vi "log.vi"(8 "error in (no error)":errorcluster, 10 "log_entry":T1 {"datetime" format="%<%x %.3X>T"}, 11 "json.provider in":refnum<class "json.provider.lvclass">) -> (0 "error out":errorcluster, 3 "json.provider out":refnum<class "json.provider.lvclass">)   [LabVIEW 2021, in "json.provider.lvclass"]
uses:
  json.provider.lvclass
  Z:/Projects/PCCS/labview-system-logging/source/system.logging.provider/system.logging.provider.lvclass
  system.logging/log_entry.ctl
  system.logging/severity.ctl
  system.logging.provider.lvclass/system.logging.provider.ctl
  json.provider.lvclass/json.provider.ctl
  system.logging/system.logging.lvclass
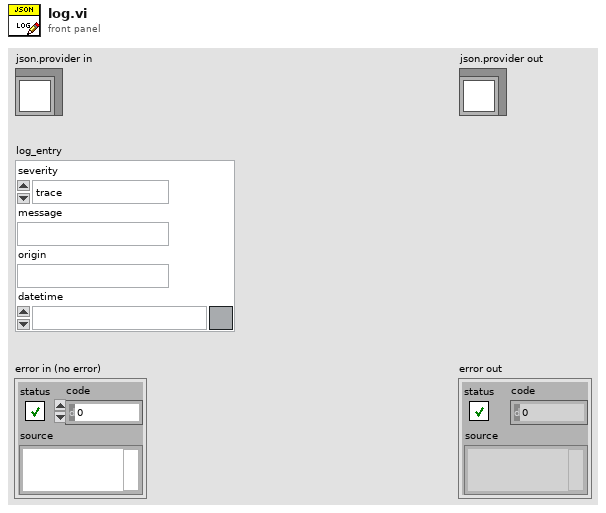
[diagram p1: front panel]
types:
  T1 = typedef "system.logging.lvclass/log_entry.ctl" = cluster{"severity":T2, "message":string, "origin":string, "datetime":timestamp}
  T2 = typedef "system.logging.lvclass/severity.ctl" = enum8{"trace", "debug", "info", "warning", "error"}
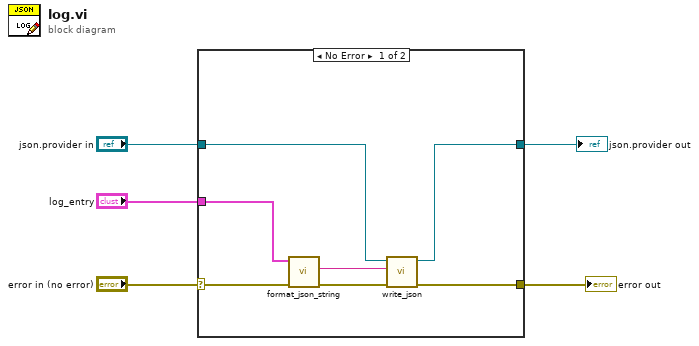
[diagram p0: block diagram]
diagram:
  n1 = case shown="No Error" "error in (no error)" {
    selector: "error in (no error)" -> [w7 w14]
    tunnel: [w12 w14] -> w2
    tunnel: [w11 w13] -> w1
    tunnel: "json.provider in" -> [w6 w13]
    tunnel: "log_entry" -> [w10 _]
    frame No Error {
      n2 = call "format_json_string.vi"("error in (no error)"=w7, "log_entry"=w10) -> ("error out"=w9:errorcluster, "json"=w8:string)  [unwired: 8 in]
      n3 = call "write_json.vi"("error in (no error)"=w9, "json"=w8, "json.provider in"=w6) -> ("error out"=w12:errorcluster, "json.provider out"=w11:refnum<class "json.provider.lvclass">)  [unwired: 7 in]
    }
    frame Error {
    }
  }
  "error out" <- w2
  "json.provider out" <- w1
